vi "Plot Bezier Spline.vi"() -> ()   [LabVIEW 2020]
panel:
  out "ctrl pts":cluster{sgl, sgl}[][](array[cluster])
  out "l total 2":dbl
  out "bezier spline":cluster{"x":dbl, "y":dbl}[](array[cluster])
  out "Spline Graph 2":cluster{"x":sgl, "y":sgl}[](graph)
  out "Waveform Graph 3":dbl[](graph)
  out "Waveform Graph 2":dbl[](graph)
  out "Waveform Graph":dbl[](graph)
  in  "Limits":T1={"Velocity (fps)"=5.0, "Accel (fps^2)"=10.0, "Jerk (fps^3)"=100.0}
  out "l total":dbl
  out "l":dbl[](array[numeric])
  in  "ending orientation":dbl=nan
  out "curvature time":u32
  out "Spline Graph":cluster{"curve ":cluster{"x":dbl, "y":dbl}[]}[](graph)
  out "Curvature":dbl[](graph)
  out "spline time":u32
  in  "percision":dbl=0.01
  in  "starting orientation":dbl
  in  "waypoints":cluster{dbl, dbl}[](array[cluster])
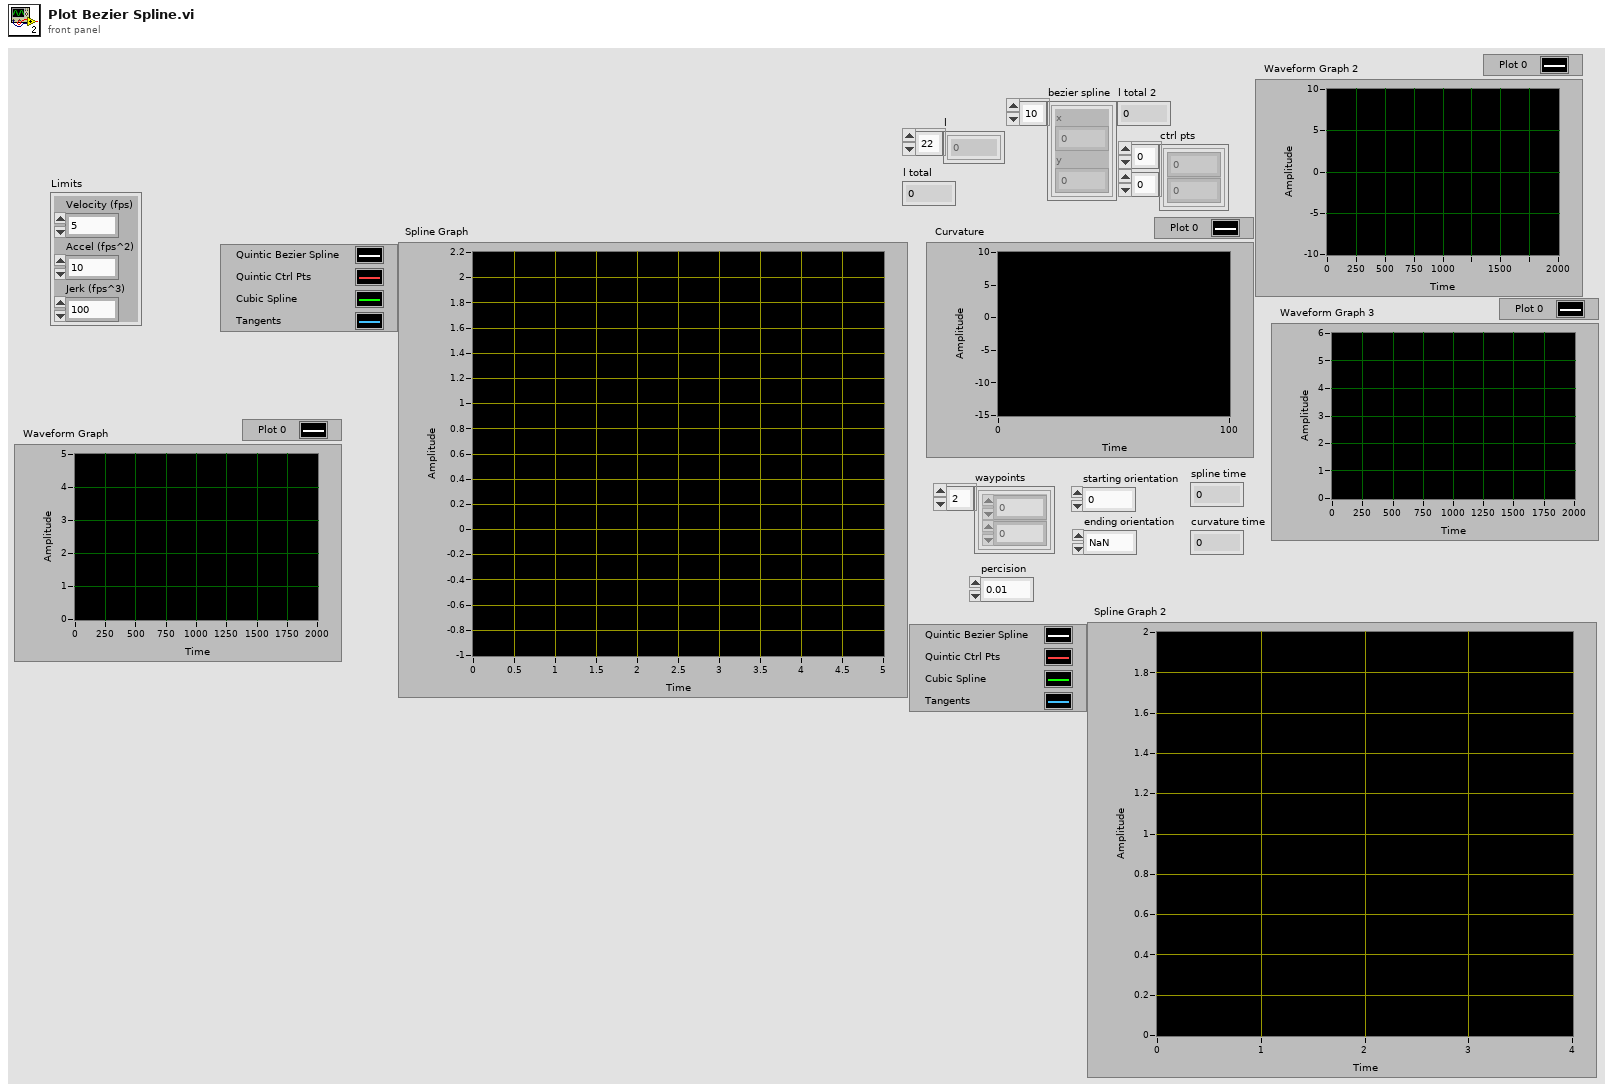
[diagram p1: front panel]
types:
  T1 = cluster{"Velocity (fps)":dbl, "Accel (fps^2)":dbl, "Jerk (fps^3)":dbl}
  T2 = typedef "Bezier Curve.ctl" = cluster{"x":sgl, "y":sgl}[]
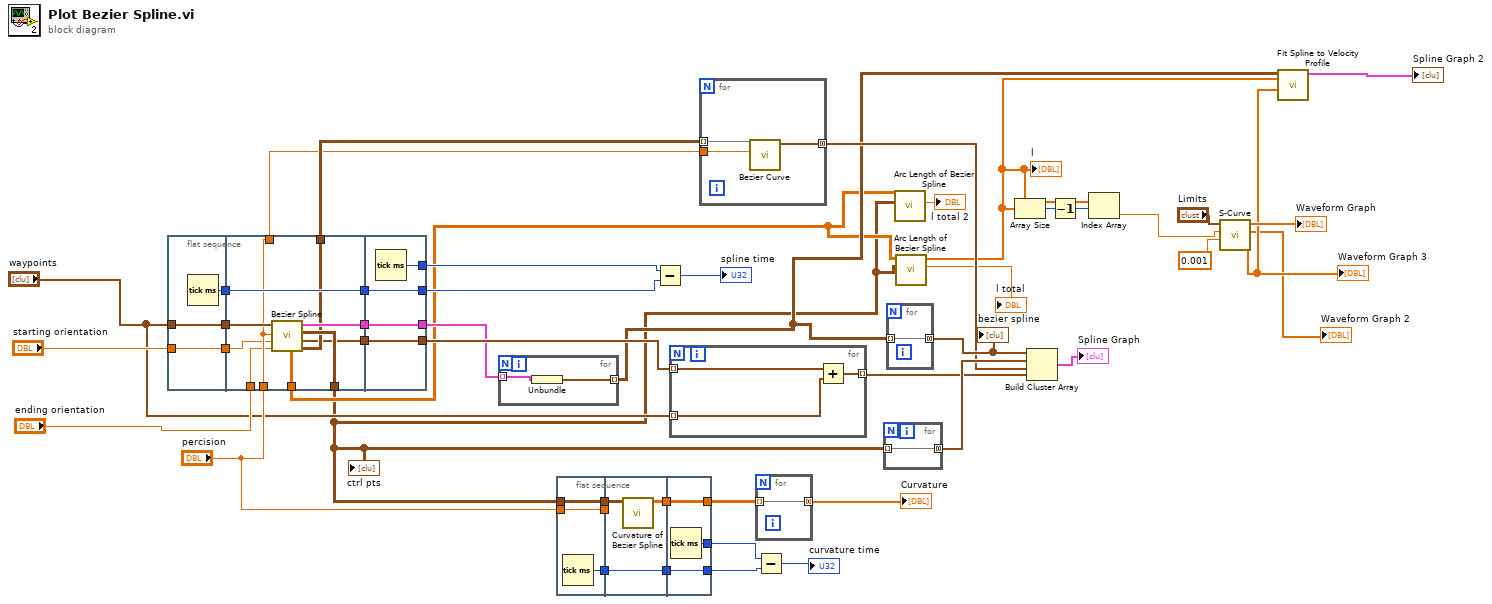
[diagram p0: block diagram]
diagram:
  n1 = flat-sequence {
    tunnel: [w50] -> w44
    tunnel: [w49] -> w42
    tunnel: "waypoints" -> [w49]
    tunnel: [w48] -> w41
    tunnel: "starting orientation" -> [w48]
    tunnel: [w60] -> w45
    tunnel: w44 -> [w60]
    tunnel: w42 -> [w59]
    tunnel: w41 -> [w53]
    tunnel: "percision" -> [w54]
    tunnel: [w58] -> w39
    tunnel: [w57] -> w2
    tunnel: [w56] -> w33
    tunnel: [w54] -> w32
    tunnel: [w55] -> w21
    tunnel: "ending orientation" -> [w52]
    tunnel: [w51] -> w3
    tunnel: [w64] -> w47
    tunnel: [w63] -> w46
    tunnel: w45 -> [w63]
    tunnel: [w62] -> w5
    tunnel: w39 -> [w62]
    tunnel: [w61] -> w10
    tunnel: w21 -> [w61]
    frame #0 {
      n2 = Tick Count (ms)() -> (millisecond timer value=w50:u32)
    }
    frame #1 {
      n3 = call "Bezier Spline.vi"("ending orientation"=w52, "starting orientation"=w53, "percision"=w54, "waypts"=w59) -> ("cubic spline ctrl pts"=w56:cluster{sgl, sgl}[][], "Tangents"=w55:cluster{sgl, sgl}[], "ctrl pts"=w57:cluster{sgl, sgl}[][], "bezier spline"=w58:cluster{"curve ":T2}[], "position out"=w51:sgl[][])  [unwired: 3 in]
    }
    frame #2 {
      n4 = Tick Count (ms)() -> (millisecond timer value=w64:u32)
    }
  }
  n5 = for {
    tunnel: w5 -> [w66] mode=indexing
    tunnel: [w65] -> w4 mode=indexing
    n6 = Unbundle(w66) -> ("curve"=w65:T2)
  }
  n7 = flat-sequence {
    tunnel: w2 -> [w68]
    tunnel: "percision" -> [w69]
    tunnel: [w69] -> w28
    tunnel: [w68] -> w27
    tunnel: [w67] -> w23
    tunnel: [w72] -> w29
    tunnel: w28 -> [_]
    tunnel: w27 -> [w71]
    tunnel: [w70] -> w24
    tunnel: w23 -> [w70]
    tunnel: [w75] -> w37
    tunnel: w29 -> [w75]
    tunnel: [w74] -> w26
    tunnel: [w73] -> w25
    tunnel: w24 -> [w73]
    frame #0 {
      n8 = Tick Count (ms)() -> (millisecond timer value=w67:u32)
    }
    frame #1 {
      n9 = call "Curvature of Bezier Spline.vi"("bezier spline waypts"=w71) -> ("curvature"=w72:dbl[][])  [unwired: 10 in]
    }
    frame #2 {
      n10 = Tick Count (ms)() -> (millisecond timer value=w74:u32)
    }
  }
  n11 = Subtract(x=w47, y=w46) -> (x-y=→"spline time":u32)
  n12 = for {
    tunnel: w10 -> [w78] mode=indexing
    tunnel: [w77] -> w9 mode=indexing
    tunnel: "waypoints" -> [w76] mode=indexing
    n13 = Add(x=w78, y=w76) -> (x+y=w77:cluster{dbl, dbl})
  }
  n14 = for {
    tunnel: w33 -> [w81] mode=indexing
    tunnel: w32 -> [w80]
    tunnel: [w79] -> w31 mode=concatenating
    n15 = call "Bezier Curve.vi"("percision"=w80, "ctrl points"=w81) -> ("curve"=w79:T2)  [unwired: 8 in, 1 out]
  }
  n16 = for {
    tunnel: [w82] -> w30 mode=concatenating
    tunnel: w37 -> [w82] mode=indexing
  }
  "Curvature" <- w30
  n17 = Subtract(x=w26, y=w25) -> (x-y=→"curvature time":u32)
  n18 = for {
    tunnel: [w83] -> w35 mode=concatenating
    tunnel: w2 -> [w83] mode=indexing
  }
  n19 = for {
    tunnel: w4 -> [w84] mode=indexing
    tunnel: [w84] -> w36 mode=concatenating
  }
  "bezier spline" <- w36
  n20 = call "Arc Length of Bezier Spline.vi"("ctrl pts"=w2, "position"=w3) -> ("l total"=→"l total 2":dbl)  [unwired: 6 in, 3 out]
  n21 = call "Arc Length of Bezier Spline.vi"("ctrl pts"=w2, "position"=w3) -> ("l total"=→"l total":dbl, "l"=w12:dbl[])  [unwired: 6 in, 2 out]
  "l" <- w12
  n22 = Array Size(array=w12) -> (size(s)=w14:i32)
  n23 = Build Cluster Array(w36, w35, w31, w9) -> (→"Spline Graph":cluster{"curve ":cluster{"x":dbl, "y":dbl}[]}[])
  n24 = Decrement(x=w14) -> (x-1=w13:i32)
  n25 = Index Array(array=w12, index=w13) -> (element=w11:dbl)
  n26 = call "S-Curve.vi"("dt (s)"=0.001, "goal"=w11, "Limits"="Limits") -> ("X"=w16:dbl[], "A"=→"Waveform Graph 2":dbl[], "V"=→"Waveform Graph":dbl[])  [unwired: 5 in, 1 out]
  "Waveform Graph 3" <- w16
  n27 = call "Fit Spline to Velocity Profile.vi"("vel positions"=w16, "s(t)"=w12, "t flat"=w4) -> ("y unflat"=→"Spline Graph 2":cluster{dbl[]}[])  [unwired: 7 in, 1 out]
  "ctrl pts" <- w2
